vi "GetInheritance.vi"(0 "ClassReaderNative in":refnum<class "ClassReaderNative.lvclass">, 5 "error in (no error)":errorcluster) -> (14 "ClassReaderNative out":refnum<class "ClassReaderNative.lvclass">, 15 "Inheritance":path[](array[path]), 16 "Inherits":bool, 19 "error out":errorcluster)   [LabVIEW 2020, in "ClassReaderNative.lvclass"]
uses:
  ClassReaderNative.lvclass
  ClassReaderNative.lvclass/ClassReaderNative.ctl
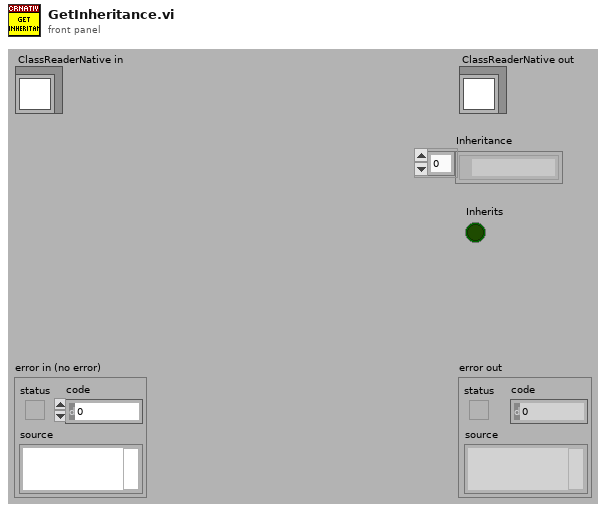
[diagram p1: front panel]
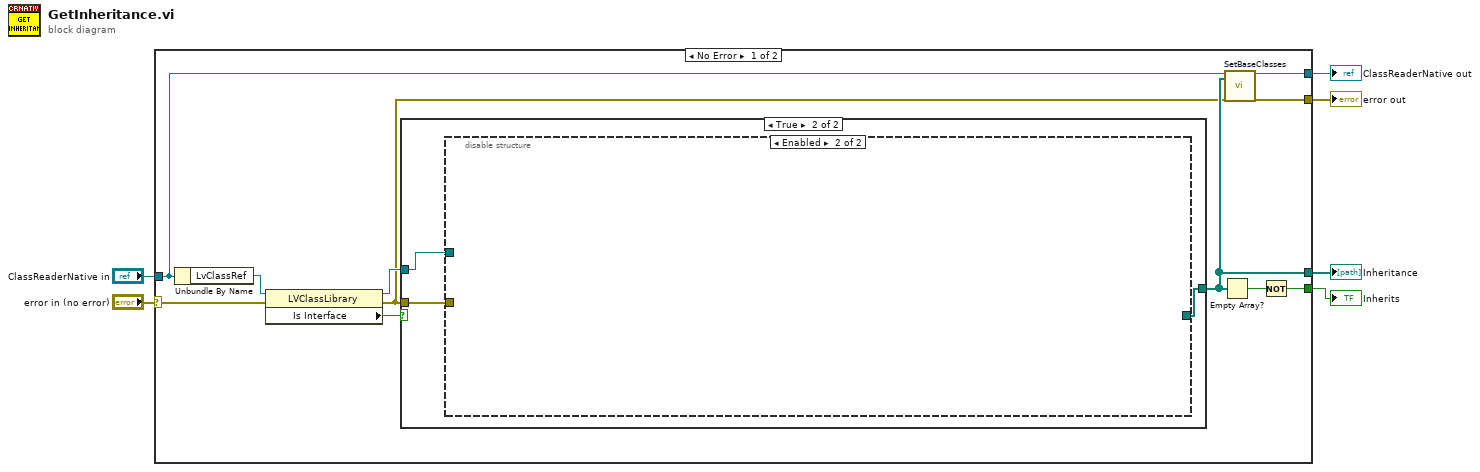
[diagram p0: block diagram]
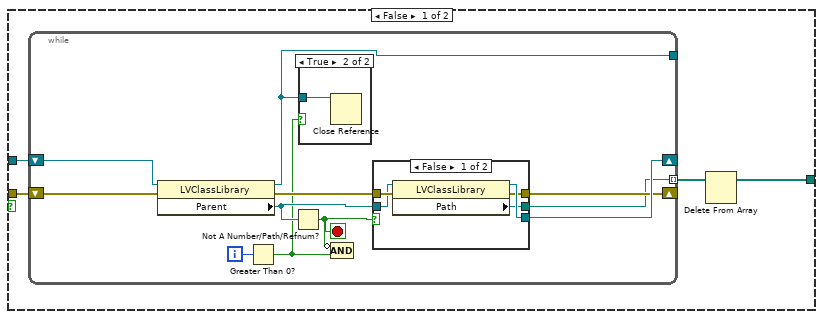
[diagram p2: hidden frame]
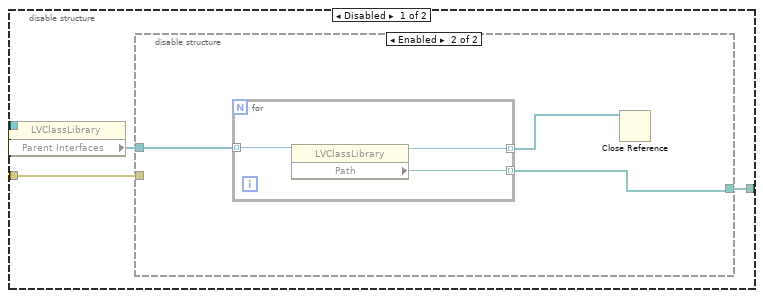
[diagram p5: hidden frame]
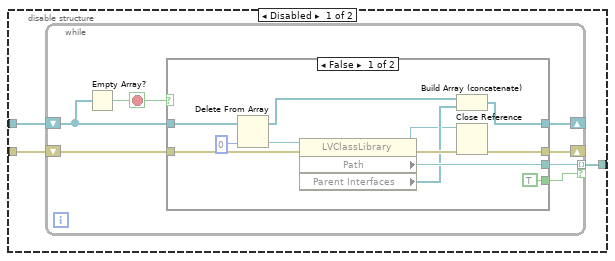
[diagram p6: hidden frame]
diagram:
  n1 = case shown="No Error" "error in (no error)" {
    selector: "error in (no error)" -> [w9 w78]
    tunnel: [w14 _] -> w6
    tunnel: [w16 _] -> w5
    tunnel: "ClassReaderNative in" -> [w13 w77]
    tunnel: [w15 w78] -> w2
    tunnel: [w7 w77] -> w1
    frame No Error {
      n2 = Unbundle By Name(w13) -> ("LvClassRef"=w12:refnum<vi>)
      n3 = property class="LVClassLibrary"(reference=w12, error in=w9) -> (reference out=w11:refnum<vi>, error out=w8:errorcluster, "Is Interface"=w10:bool)
      n4 = case shown="True" w10 {
        tunnel: [w20 w41] -> w14
        tunnel: w8 -> [w19 w43]
        tunnel: w11 -> [w18 w42]
        frame False {
          n5 = while {
            shift-right: [w28] -> _
            shift-left: w18 -> [w32]
            tunnel: [w30] -> _
            shift-right: [w26] -> _
            shift-left: w19 -> [w31]
            tunnel: [w25] -> w21 mode=indexing
            i -> [w29]
            stop <- w23 stop-if-true
            n6 = property class="LVClassLibrary"(reference=w32, error in=w31) -> (reference out=w30:refnum<vi>, error out=w27:errorcluster, "Parent"=w24:refnum<vi>)
            n7 = Greater Than 0?(x=w29) -> (x > 0?=w22:bool)
            n8 = Not A Number/Path/Refnum?(number/path/refnum=w24) -> (NaN/Path/Refnum?=w23:bool)
            n9 = case shown="True" w22 {
              tunnel: w30 -> [_ w40]
              frame False {
              }
              frame True {
                n10 = Close Reference(reference=w40) -> ()  [unwired: 1 in, 1 out]
              }
            }
            n11 = Compound Arithmetic op=AND(invert w23, w22) -> ()  [unwired: 1 out]
            n12 = case shown="False" w23 {
              tunnel: [w37 w38] -> w28
              tunnel: w27 -> [w36 w39]
              tunnel: [w35 w39] -> w26
              tunnel: [w34 _] -> w25
              tunnel: w24 -> [w33 w38]
              frame False {
                n13 = property class="LVClassLibrary"(reference=w33, error in=w36) -> (reference out=w37:refnum<vi>, error out=w35:errorcluster, "Path"=w34:path)
              }
              frame True {
              }
            }
          }
          n14 = Delete From Array(array=w21) -> (array with subset deleted=w20:path[])  [unwired: 2 in, 1 out]
        }
        frame True {
          n15 = disable-structure shown="Enabled" {
            disable-tunnel: w43 -> [w47 _]
            disable-tunnel: w42 -> [w46 _]
            disable-tunnel: [w44 _] -> w41
            frame Disabled {
              n16 = property class="LVClassLibrary"(reference=w46) -> ("Parent Interfaces"=w45:refnum<vi>[])  [unwired: 1 in, 2 out]
              n17 = disable-structure shown="Enabled" {
                disable-tunnel: w47 -> [w50 _]
                disable-tunnel: w45 -> [w49 w73]
                disable-tunnel: [w48 w72] -> w44
                frame Disabled {
                  n18 = while {
                    shift-right: [w51] -> _
                    shift-left: w49 -> [w52]
                    shift-right: [w57] -> _
                    shift-left: w50 -> [w55]
                    tunnel: [w56] -> w48 mode=indexing if=w54
                    stop <- w53 stop-if-true
                    n19 = Empty Array?(array=w52) -> (empty?=w53:bool)
                    n20 = case shown="False" w53 {
                      tunnel: w55 -> [w69 w70]
                      tunnel: [w66 w70] -> w57
                      tunnel: [w68 _] -> w56
                      tunnel: [TRUE _] -> w54
                      tunnel: w52 -> [w64 _]
                      tunnel: [w61 _] -> w51
                      frame False {
                        n21 = Delete From Array(array=w64, index=0) -> (deleted portion=w63:refnum<vi>, array with subset deleted=w60:refnum<vi>[])  [unwired: 1 in]
                        n22 = property class="LVClassLibrary"(reference=w63, error in=w69) -> (reference out=w58:refnum<vi>, error out=w67:errorcluster, "Path"=w68:path, "Parent Interfaces"=w62:refnum<vi>[])
                        n23 = Build Array (concatenate)(w60, w62) -> (w61:refnum<vi>[])
                        n24 = Close Reference(reference=w58, error in (no error)=w67) -> (error out=w66:errorcluster)
                      }
                      frame True {
                      }
                    }
                  }
                }
                frame Enabled {
                  n25 = for {
                    tunnel: w73 -> [w76] mode=indexing
                    tunnel: [w75] -> w72 mode=indexing
                    tunnel: [w74] -> w71 mode=indexing
                    n26 = property class="LVClassLibrary"(reference=w76) -> (reference out=w74:refnum<vi>, "Path"=w75:path)  [unwired: 1 in, 1 out]
                  }
                  n27 = Close Reference(reference=w71) -> ()  [unwired: 1 in, 1 out]
                }
              }
            }
            frame Enabled {
            }
          }
        }
      }
      n28 = Empty Array?(array=w14) -> (empty?=w17:bool)
      n29 = call-dynamic "SetBaseClasses.vi"("ClassReader in"=w13, "Inheritance"=w14, "error in (no error)"=w8) -> ("ClassReader out"=w7:refnum<class "ClassReaderNative.lvclass">, "error out"=w15:errorcluster)  [unwired: 15 in]
      n30 = Not(x=w17) -> (.not. x?=w16:bool)
    }
    frame Error {
    }
  }
  "ClassReaderNative out" <- w1
  "Inheritance" <- w6
  "Inherits" <- w5
  "error out" <- w2
